vi "to string.vi"(8 "error in":errorcluster, 11 "engine configuration in":refnum<class "engine configuration.lvclass">) -> (0 "error out":errorcluster, 1 "data":string, 2 "version":string, 3 "engine configuration out":refnum<class "engine configuration.lvclass">)   [LabVIEW 2014, in "engine configuration.lvclass"]
doc: "This VI takes an Engine Configuration object and flattens it into a string with corresponding version. The version is used that the data string can be unflattenend successfully as the configuration object evolves over time."
uses:
  engine configuration.lvclass
  engine configuration.lvclass/engine configuration.ctl
  <vilib>/NI/Tag Bus Module Framework/root configuration/TBM configuration.lvclass
  <vilib>/NI/Configuration Framework/serializable configuration/NISE_CEF_serializable configuration.lvclass
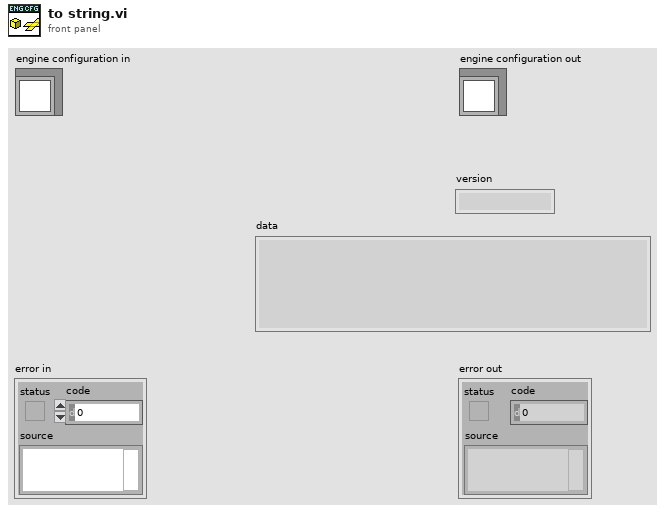
[diagram p1: front panel]
types:
  T1 = typedef "engine configuration.lvclass/module channel pairings.ctl" = cluster{"modules":string[], "channels":string[]}
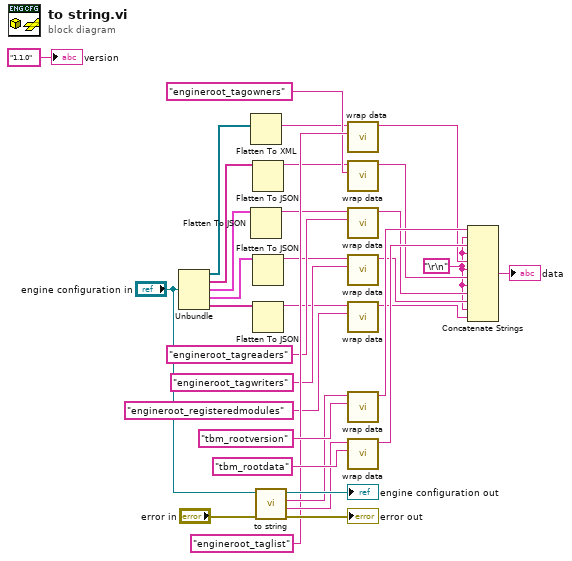
[diagram p0: block diagram]
diagram:
  w9 = "\r\n"
  n1 = Unbundle("engine configuration in") -> (w2:refnum<class "tag descriptor.lvclass">[], w8:string[], w17:T1[], w6:T1, w4:string[])
  n2 = Flatten To XML(anything=w2) -> (xml string=w1:string)
  n3 = Flatten To JSON(anything=w17) -> (JSON string=w15:string)  [unwired: 2 in, 1 out]
  n4 = Flatten To JSON(anything=w8) -> (JSON string=w7:string)  [unwired: 2 in, 1 out]
  n5 = Flatten To JSON(anything=w6) -> (JSON string=w5:string)  [unwired: 2 in, 1 out]
  n6 = Flatten To JSON(anything=w4) -> (JSON string=w3:string)  [unwired: 2 in, 1 out]
  n7 = call-parent "to string.vi"("error in"="error in", "configuration in"="engine configuration in") -> ("error out"=→"error out":errorcluster, "data"=w25:string, "version"=w26:string, "configuration out"=→"engine configuration out":refnum<class "engine configuration.lvclass">)  [unwired: 6 in]
  n8 = call <vilib>:"wrap data.vi"("identifier"="engineroot_taglist" ("additional identifier"), "data to wrap"=w1) -> ("wrapped data"=w20:string)  [unwired: 9 in]
  n9 = call <vilib>:"wrap data.vi"("identifier"="engineroot_tagowners" ("additional identifier"), "data to wrap"=w7) -> ("wrapped data"=w19:string)  [unwired: 9 in]
  n10 = call <vilib>:"wrap data.vi"("identifier"="engineroot_tagreaders" ("additional identifier"), "data to wrap"=w15) -> ("wrapped data"=w14:string)  [unwired: 9 in]
  n11 = call <vilib>:"wrap data.vi"("identifier"="engineroot_tagwriters" ("additional identifier"), "data to wrap"=w5) -> ("wrapped data"=w10:string)  [unwired: 9 in]
  n12 = call <vilib>:"wrap data.vi"("identifier"="engineroot_registeredmodules" ("additional identifier"), "data to wrap"=w3) -> ("wrapped data"=w11:string)  [unwired: 9 in]
  n13 = call <vilib>:"wrap data.vi"("identifier"="tbm_rootversion" ("additional identifier"), "data to wrap"=w26) -> ("wrapped data"=w27:string)  [unwired: 9 in]
  n14 = call <vilib>:"wrap data.vi"("identifier"="tbm_rootdata" ("additional identifier"), "data to wrap"=w25) -> ("wrapped data"=w28:string)  [unwired: 9 in]
  n15 = Concatenate Strings(w27, w9, w28, w9, w20, w9, w19, w9, w14, w10, w9, w11) -> (→"data":string)
  "version" <- "1.1.0" ("Version")
